vi "libssh2_init.vi"   [LabVIEW 2017, in "libssh2.lvlib"]
doc: "Initialize libssh2."
uses:
  libssh2.lvlib
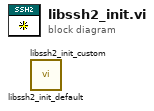
[diagram p0: block diagram]
diagram:
  n1 = call "libssh2_init_default.vi"() -> ()  [unwired: 11 in, 1 out]
  n2 = call "libssh2_init_custom.vi"() -> ()  [unwired: 11 in, 1 out]
